vi "Read reference.vi"(8 "error in (no error)":errorcluster, 11 "ToastService in":refnum<class "ToastService.lvclass">) -> (0 "error out":errorcluster, 2 "reference":refnum<k24>, 3 "ToastService out":refnum<class "ToastService.lvclass">)   [LabVIEW 2026, in "ToastNotification.lvlib" / "ToastService.lvclass"]
doc: "Native data-member read accessor for the notification manager reference. The output is a borrowed alias; no native object is created or closed. Pass the class and error through. The service owns its native reference lifetime."
uses:
  ToastService.lvclass
  C:/Users/loicw/Documents/LabVIEW/ToastNotifications/Sources/bins/Microsoft.Toolkit.Uwp.Notifications.dll
  bins/Microsoft.Toolkit.Uwp.Notifications.dll
  ToastService.lvclass/ToastService.ctl
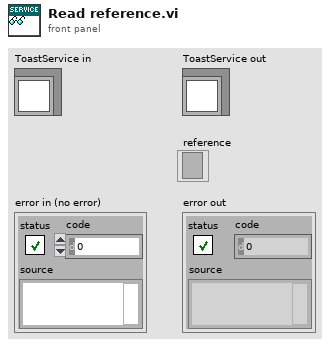
[diagram p1: front panel]
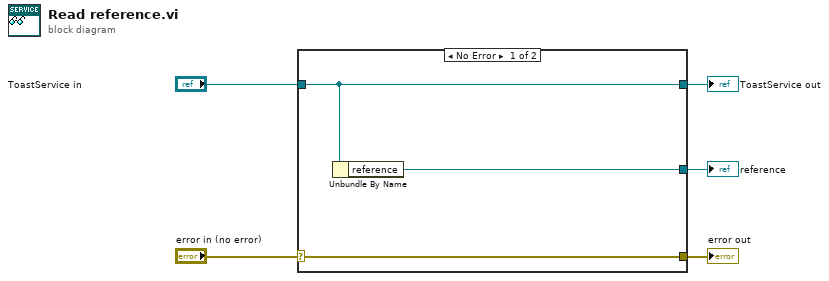
[diagram p0: block diagram]
diagram:
  n1 = case shown="No Error" "error in (no error)" {
    selector: "error in (no error)" -> [w8 w9]
    tunnel: [w8 w9] -> w4
    tunnel: [w7 w10] -> w2
    tunnel: "ToastService in" -> [w7 w10]
    tunnel: [w6 _] -> w1
    frame No Error {
      n2 = Unbundle By Name(w7) -> ("reference"=w6:refnum<k24>)
    }
    frame Error {
    }
  }
  "error out" <- w4
  "ToastService out" <- w2
  "reference" <- w1
